vi "Destroy Test Assert Factory.vi"(6 "register caller level (0)":i32, 8 "error in (no error)":errorcluster, 11 "Test Assert Factory in":refnum<class "Test Assert Factory.lvclass">) -> (0 "error out":errorcluster)   [LabVIEW 2020, in "Caraya.lvlib" / "Test Assert Factory.lvclass"]
uses:
  Test Assert Factory.lvclass
  Test Assert Factory.lvclass/Test Assert Factory.ctl
  Test Result/Test Result.lvclass
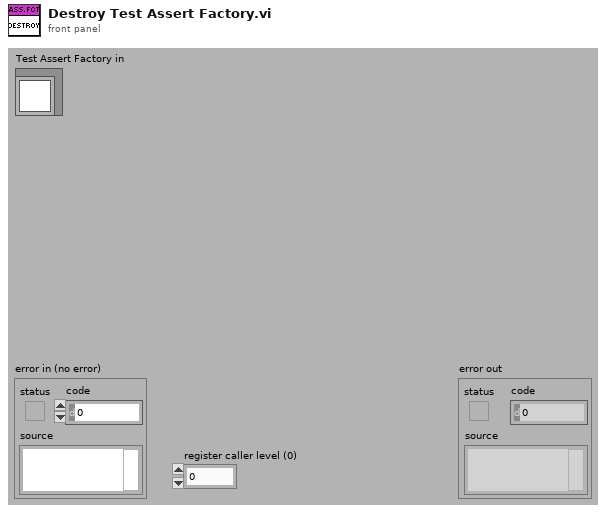
[diagram p1: front panel]
types:
  T1 = typedef "Caraya.lvlib/Test Result.lvclass/Test Events -- cluster.ctl" = cluster{"Test Registration Event":refnum<user-event>, "Assertion Event":refnum<user-event>, "Assertion Update Event":refnum<user-event>}
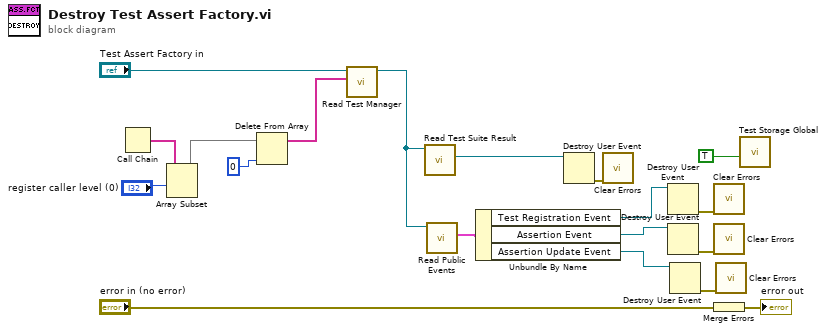
[diagram p0: block diagram]
diagram:
  n1 = Call Chain() -> (call chain=w3:string[])
  n2 = Array Subset(array=w3, index="register caller level (0)") -> (w2:string[])  [unwired: 1 in]
  n3 = Delete From Array(array=w2, index=0) -> (array with subset deleted=w15:string[])  [unwired: 1 in, 1 out]
  n4 = call-dynamic "Read Test Manager.vi"("VI Call Chain"=w15, "Assert Factory in"="Test Assert Factory in") -> ("Assert Factory out"=w12:refnum<class "Test Assert Factory.lvclass">)  [unwired: 7 in, 2 out]
  n5 = call "Read Test Suite Result.vi"("Test Assert Factory in"=w12) -> ("Test Suite Result"=w14:refnum<user-event>)  [unwired: 8 in, 2 out]
  n6 = call "Read Public Events.vi"("Test Assert Factory in"=w12) -> ("Public Events"=w11:T1)  [unwired: 8 in, 2 out]
  n7 = Unbundle By Name(w11) -> ("Test Registration Event"=w9:refnum<user-event>, "Assertion Event"=w7:refnum<user-event>, "Assertion Update Event"=w5:refnum<user-event>)
  n8 = Destroy User Event(user event=w14) -> (error out=w13:errorcluster)  [unwired: 1 in]
  n9 = call <vilib>:"Clear Errors.vi"("error in (no error)"=w13) -> ()  [unwired: 5 in, 2 out]
  n10 = Destroy User Event(user event=w9) -> (error out=w10:errorcluster)  [unwired: 1 in]
  n11 = Destroy User Event(user event=w7) -> (error out=w8:errorcluster)  [unwired: 1 in]
  n12 = Destroy User Event(user event=w5) -> (error out=w6:errorcluster)  [unwired: 1 in]
  n13 = call <vilib>:"Clear Errors.vi"("error in (no error)"=w10) -> ()  [unwired: 5 in, 2 out]
  n14 = call <vilib>:"Clear Errors.vi"("error in (no error)"=w8) -> ()  [unwired: 5 in, 2 out]
  n15 = Merge Errors("error in (no error)") -> (→"error out":errorcluster)
  n16 = call <vilib>:"Clear Errors.vi"("error in (no error)"=w6) -> ()  [unwired: 5 in, 2 out]
  n17 = call "Test Storage Global.vi"("Clear (F)"=TRUE) -> ()  [unwired: 7 in, 4 out]
